vi "angle_monitor.vi"() -> ()   [LabVIEW 2020]
uses:
  <vilib>/xnet/xnet.llb/XNET Create Session (Frame Input Stream).vi
  <vilib>/xnet/xnet.llb/XNET Read (Frame CAN).vi
  PlotGraph.llb/Plot_Y_Graph(RelativeTime-Scope).vi
  <resource>/objmgr/xnet.rc
  PlotGraph.llb/GraphPlot.lvlib
panel:
  out "XY Graph":cluster{dbl[], dbl[]}[](graph)
  in  "stop":bool
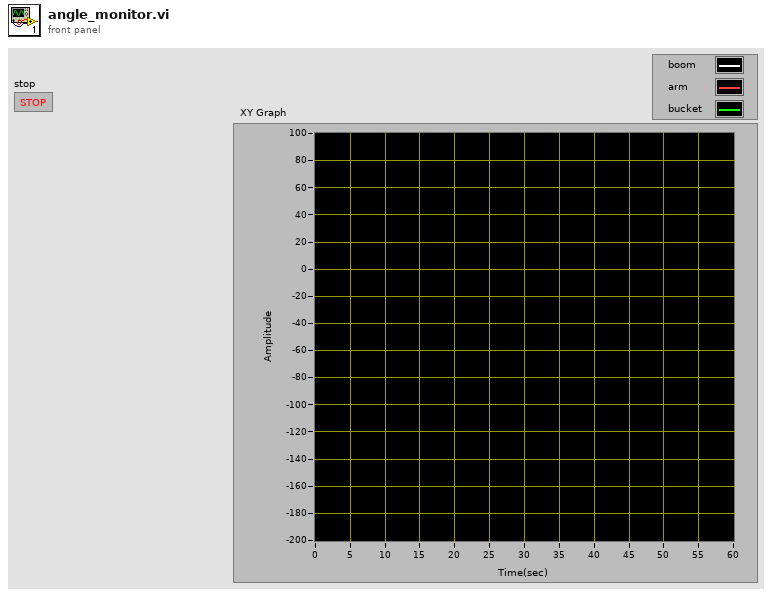
[diagram p1: front panel]
types:
  T1 = typedef "XNET Frame CAN.ctl" = cluster{"timestamp":timestamp, "payload":u8[], "identifier":u32, "type":T2, "extended?":bool, "echo?":bool}
  T2 = typedef "XNET Frame Type CAN.ctl" = u8
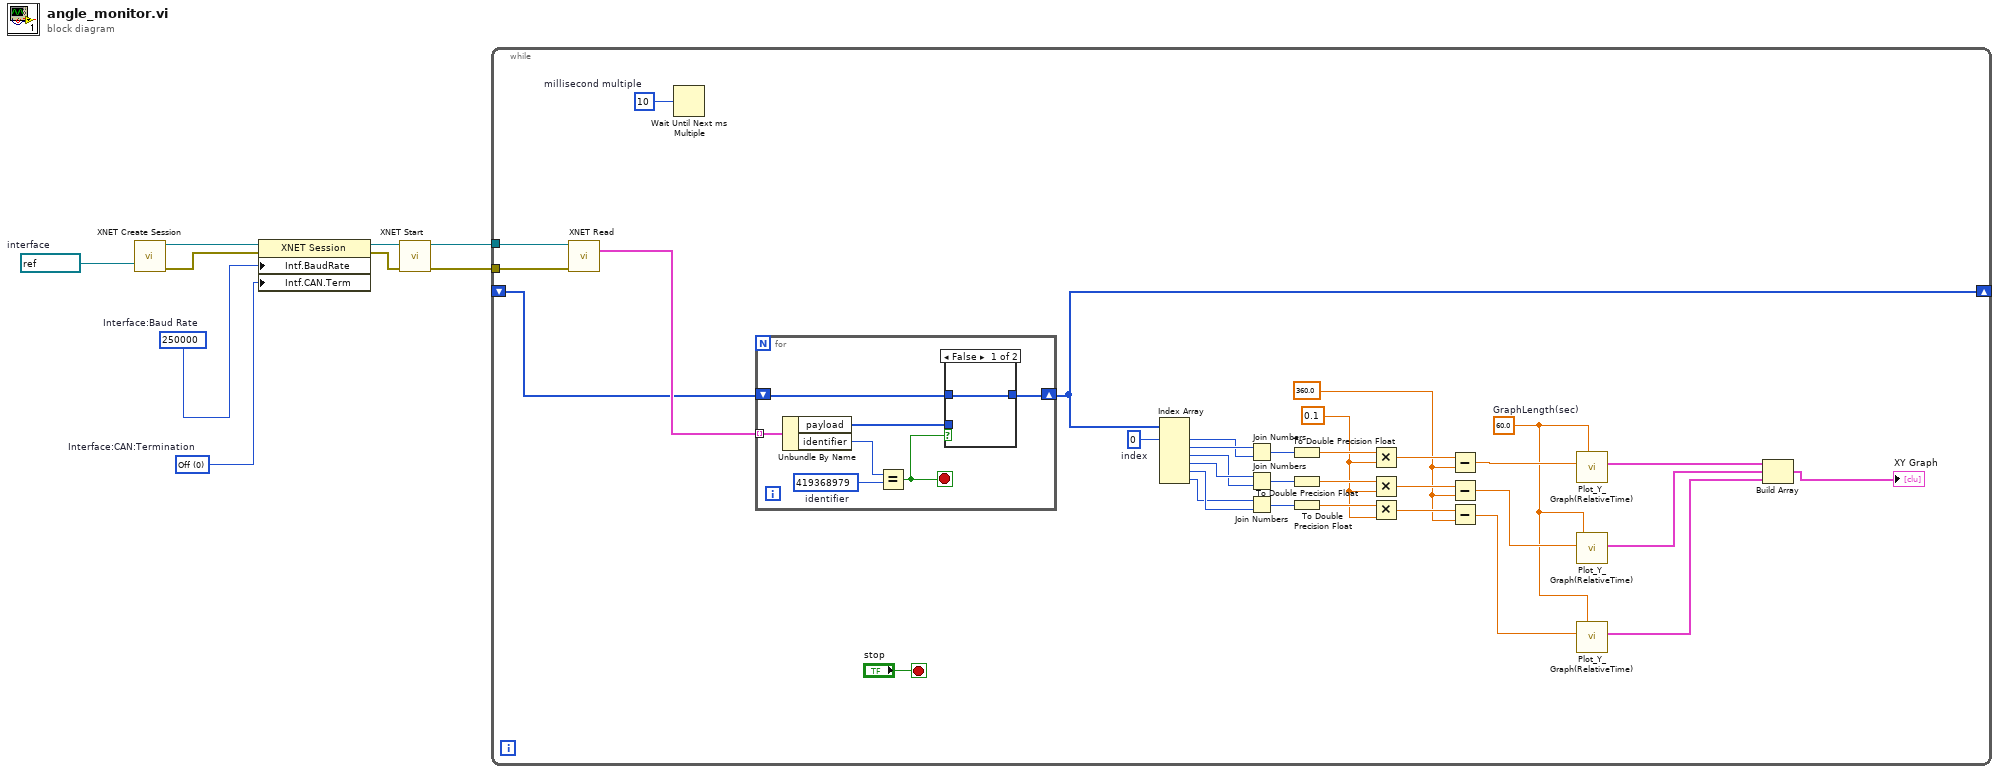
[diagram p0: block diagram]
diagram:
  w1 = u32 0 items=["Off", "On"]  # Interface:CAN:Termination
  w4 = u32 250000  # Interface:Baud Rate
  w9 = refnum<k21> "CAN1"  # interface
  n1 = call-poly <vilib>:"XNET Create Session.vi"("interface"=w9) -> ("session out"=w8:refnum<k21>, "error out"=w3:errorcluster)  [unwired: 13 in]
  n2 = property class="XNET Session"(reference=w8, error in=w3, "Intf.BaudRate"=w4, "Intf.CAN.Term"=w1) -> (reference out=w5:refnum<k21>, error out=w2:errorcluster)
  n3 = call <vilib>:"XNET Start.vi"("session in"=w5, "error in (no error)"=w2) -> ("session out"=w7:refnum<k21>, "error out"=w6:errorcluster)  [unwired: 12 in]
  n4 = while {
    tunnel: w7 -> [w42]
    tunnel: w6 -> [w41]
    shift-right: [w18] -> _
    shift-left: _ -> [w19]
    stop <- "stop" stop-if-true
    w10 = 60.0  # GraphLength(sec)
    w20 = 360.0
    w24 = 0.1
    w37 = 0  # index
    w39 = u32 10  # millisecond multiple
    n5 = call-poly <vilib>:"XNET Read.vi"("session in"=w42, "error in (no error)"=w41) -> ("data"=w38:T1[])  [unwired: 10 in, 3 out]
    n6 = Wait Until Next ms Multiple(millisecond multiple=w39) -> ()  [unwired: 1 out]
    n7 = for {
      tunnel: w38 -> [w49] mode=indexing
      shift-right: [w45] -> w18
      shift-left: w19 -> [w43]
      stop <- w46 stop-if-true
      w48 = u32 419368979  # identifier
      n8 = Unbundle By Name(w49) -> ("payload"=w44:u8[], "identifier"=w47:u32)
      n9 = Equal?(x=w47, y=w48) -> (x = y?=w46:bool)
      n10 = case shown="False" w46 {
        tunnel: [w50 w51] -> w45
        tunnel: w44 -> [_ w51]
        tunnel: w43 -> [w50 _]
        frame False {
        }
        frame True {
        }
      }
    }
    n11 = Index Array(array=w18, index #1=w37) -> (element #1=w35:u8, element #2=w36:u8, element #3=w33:u8, element #4=w34:u8, element #5=w32:u8, element #6=w31:u8)  [unwired: 5 in]
    n12 = Join Numbers(hi=w36, lo=w35) -> ((hi.lo)=w30:u16)
    n13 = Join Numbers(hi=w34, lo=w33) -> ((hi.lo)=w29:u16)
    n14 = Join Numbers(hi=w31, lo=w32) -> ((hi.lo)=w28:u16)
    n15 = To Double Precision Float(number=w30) -> (double precision float=w27:dbl)
    n16 = To Double Precision Float(number=w29) -> (double precision float=w26:dbl)
    n17 = To Double Precision Float(number=w28) -> (double precision float=w25:dbl)
    n18 = Multiply(x=w27, y=w24) -> (x*y=w23:dbl)
    n19 = Multiply(x=w26, y=w24) -> (x*y=w22:dbl)
    n20 = Multiply(x=w25, y=w24) -> (x*y=w21:dbl)
    n21 = Subtract(x=w23, y=w20) -> (x-y=w17:dbl)
    n22 = Subtract(x=w22, y=w20) -> (x-y=w16:dbl)
    n23 = Subtract(x=w21, y=w20) -> (x-y=w15:dbl)
    n24 = call-poly "Plot_Y_Graph(RelativeTime).vi"("GraphLength(sec)"=w10, "DataInput(Y-Value)"=w17) -> ("XYGraph"=w14:cluster{dbl[], dbl[]})  [unwired: 9 in]
    n25 = call-poly "Plot_Y_Graph(RelativeTime).vi"("GraphLength(sec)"=w10, "DataInput(Y-Value)"=w16) -> ("XYGraph"=w13:cluster{dbl[], dbl[]})  [unwired: 9 in]
    n26 = call-poly "Plot_Y_Graph(RelativeTime).vi"("GraphLength(sec)"=w10, "DataInput(Y-Value)"=w15) -> ("XYGraph"=w12:cluster{dbl[], dbl[]})  [unwired: 9 in]
    n27 = Build Array(w14, w13, w12) -> (→"XY Graph":cluster{dbl[], dbl[]}[])
  }
